vi "CRC_NB.vi"() -> ()   [LabVIEW 2025, in "Procotol_class.lvclass"]
uses:
  Procotol_class.lvclass
panel:
  out "CRCL":string
  out "CRCH":string
  out "CRCcode":string
  in  "CRC校验信息":T1(array[cluster])=[{"多项式模型"="X16+X15+X2+1", "宽度"=16, "多项式"=40961, "初始值"=0, "结果异或值"=0}, {"多项式模型"="X16+X15+X2+1", "宽度"=16, "多项式"=40961, "初始值"=0, "结果异或值"=65535}, {"多项式模型"="X16+X15+X2+1", "宽度"=16, "多项式"=40961, "初始值"=65535, "结果异或值"=65535}, {"多项式模型"="X16+X15+X2+1", "宽度"=16, "多项式"=40961, "初始值"=65535, "结果异或值"=0}, {"多项式模型"="X16+X12+X2+1", "宽度"=16, "多项式"=33800, "初始值"=0, "结果异或值"=0}, {"多项式模型"="X16+X12+X5+1", "宽度"=16, "多项式"=4129, "初始值"=65535, "结果异或值"=0}, {"多项式模型"="X16+X12+X2+1", "宽度"=16, "多项式"=33800, "初始值"=65535, "结果异或值"=65535}, {"多项式模型"="X16+X15+X2+1", "宽度"=16, "多项式"=4129, "初始值"=0, "结果异或值"=0}, {"多项式模型"="X16+X13+X12+X11+X10+X8+X6+X5+X2+1", "宽度"=16, "多项式"=42684, "初始值"=0, "结果异或值"=65535}] {"结果异或值" format="%.0x"; "初始值" format="%.0x"; "多项式" format="%.0x"}
  in  "枚举":T2(ring)
  in  "data":string
  out "data+CRC":string
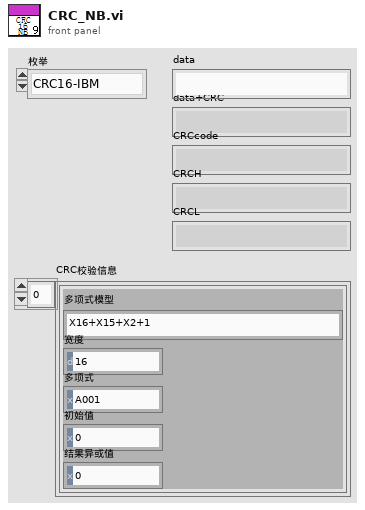
[diagram p1: front panel]
types:
  T1 = cluster{"多项式模型":string, "宽度":u16, "多项式":u16, "初始值":u16, "结果异或值":u16}[]
  T2 = enum8{"CRC16-IBM", "CRC16-MAXIM", "CRC16-USB", "CRC16-MODBUS", "CRC16-CCITT", "CRC16-CCITT-FALSE", "CRC16-X25", "CRC16-XMODEM", "CRC16-DNP"}
  T3 = cluster{"多项式模型":string, "宽度":u16, "多项式":u16, "初始值":u16, "结果异或值":u16}
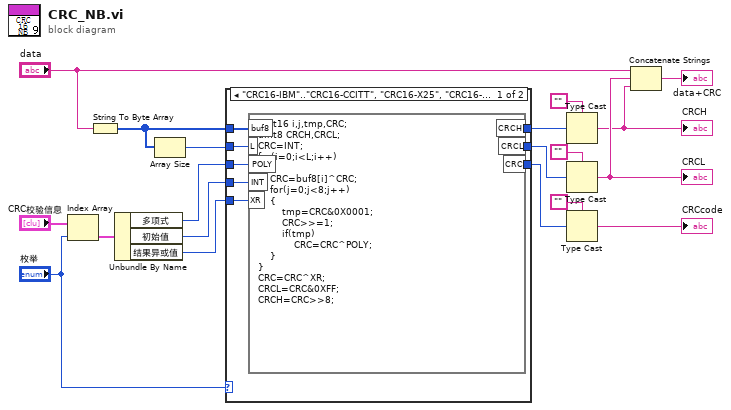
[diagram p0: block diagram]
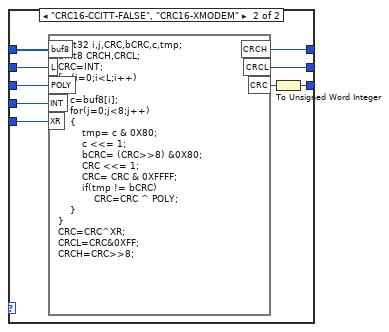
[diagram p2: hidden frame]
diagram:
  n1 = Index Array(array="CRC校验信息", index="枚举") -> (element=w13:T3)
  n2 = String To Byte Array(string="data") -> (unsigned byte array=w2:u8[])
  n3 = Unbundle By Name(w13) -> ("多项式"=w8:u16, "初始值"=w7:u16, "结果异或值"=w6:u16)
  n4 = Array Size(array=w2) -> (size(s)=w9:i32)
  n5 = case shown="\"CRC16-IBM\"..\"CRC16-CCITT\", \"CRC16-X25\", \"CRC16-DNP\"" "枚举" {
    tunnel: [w27 w30] -> w18
    tunnel: [w26 w31] -> w16
    tunnel: [w25 w29] -> w11
    tunnel: w9 -> [w24 w35]
    tunnel: w8 -> [w23 w34]
    tunnel: w7 -> [w22 w33]
    tunnel: w6 -> [w21 w32]
    tunnel: w2 -> [w20 w36]
    frame "CRC16-IBM".."CRC16-CCITT", "CRC16-X25", "CRC16-DNP" {
      n6 = formula code="uInt16 i,j,tmp,CRC;\nuInt8 CRCH,CRCL;\nCRC=INT;\nfor(i=0;i<L;i++)\n{\n    CRC=buf8[i]^CRC;\n    for(j=0;j<8;j++)\n    {\n        tmp=CRC&0X0001;\n        CRC>>=1;\n        if(tmp)\n            CRC=CRC^POLY;\n    }\n}\nCRC=CRC^XR;\nCRCL=CRC&0XFF;\nCRCH=CRC>>8;"("buf8"=w20, "L"=w24, "INT"=w22, "XR"=w21, "POLY"=w23) -> ("CRCH"=w26:u8, "CRCL"=w27:u8, "CRC"=w25:u16)
    }
    frame "CRC16-CCITT-FALSE", "CRC16-XMODEM" {
      n7 = formula code="uInt32 i,j,CRC,bCRC,c,tmp;\nuInt8 CRCH,CRCL;\nCRC=INT;\nfor(i=0;i<L;i++)\n{   \n    c=buf8[i];\n    for(j=0;j<8;j++)\n    {\n        tmp= c & 0X80;\n        c <<= 1;\n        bCRC= (CRC>>8) &0X80;\n        CRC <<= 1;\n        CRC= CRC & 0XFFFF;\n        if(tmp != bCRC)\n            CRC=CRC ^ POLY;\n    }\n}\nCRC=CRC^XR;\nCRCL=CRC&0XFF;\nCRCH=CRC>>8;"("buf8"=w36, "L"=w35, "INT"=w33, "XR"=w32, "POLY"=w34) -> ("CRC"=w28:u32, "CRCL"=w30:u8, "CRCH"=w31:u8)
      n8 = To Unsigned Word Integer(number=w28) -> (unsigned 16bit integer=w29:u16)
    }
  }
  n9 = Type Cast(type="", x=w16) -> (*(type *) &x=w4:string)
  "CRCH" <- w4
  n10 = Type Cast(type="", x=w18) -> (*(type *) &x=w5:string)
  "CRCL" <- w5
  n11 = Type Cast(type="", x=w11) -> (*(type *) &x=→"CRCcode":string)
  n12 = Concatenate Strings("data", w5, w4) -> (→"data+CRC":string)
